vi "Line Configuration Dialog.vi"(8 "error in":errorcluster, 9 "engine configuration in":refnum<class "engine configuration.lvclass">, 10 "tag bus configurable plugin module configuration":refnum<class "Daqmx Module configuration.lvclass">, 11 "Line":T5={"Channel Array"=[], "Physical Channel"="", "Measurement Type"=enum."Digital Input", "Parameters"={"Digital Config"={"Invert Lines?"=FALSE}, "Voltage Config"={"Maximum Value (V)"=5.0, "Minimum Value (V)"=-5.0, "in terminal configuration (V)"=-1, "out terminal configuration (V)"=-1}, "Current Config"={"Maximum Value (A)"=0.02, "Minimum Value (A)"=0.0, "shunt resistor location"=-1, "input terminal configuration (C)"=-1, "external shunt resistor value"=249.0}, "RTD Config"={"Maximum Value (°C)"=100.0, "Minimum Value (°C)"=0.0, "resistance configuration"=2, "r0"=100.0, "current excitation value"=0.0025, "rtd type"=10137, "current excitation source"=10167}, "Thermocouple Config"={"Minimum Value (C)"=0.0, "Maximum Value (C)"=100.0, "thermocouple type"=10072, "cjc source"=10116, "cjc value"=25.0}, "Strain Config"={"Maximum Value"=0.001, "Minimum Value"=-0.001, "bridge information"={"strain configuration"=10183, "lead wire resistance"=0.0, "initial bridge voltage"=0.0, "voltage excitation source"=10200, "voltage excitation value"=2.5}, "strain gage information"={"gage factor"=2.0, "nominal gage resistance"=350.0, "poisson ratio"=0.3}}, "PWM Config"={"Idle State"=FALSE}}} {"Parameters"."Voltage Config"."out terminal configuration (V)" items=["Default"=-1, "RSE"=10083, "Differential"=10106, "Pseudodifferential"=12529]; "Parameters"."Voltage Config"."in terminal configuration (V)" items=["Default"=-1, "RSE"=10083, "NRSE"=10078, "Differential"=10106, "Pseudodifferential"=12529]; "Parameters"."Current Config"."shunt resistor location" items=["default"=-1, "Internal"=10200, "External"=10167]; "Parameters"."Current Config"."input terminal configuration (C)" items=["default"=-1, "RSE"=10083, "NRSE"=10078, "Differential"=10106, "Pseudodifferential"=12529]; "Parameters"."RTD Config"."resistance configuration" items=["2-Wire"=2, "3-Wire"=3, "4-Wire"=4]; "Parameters"."RTD Config"."rtd type" items=["Pt3750"=12481, "Pt3851"=10071, "Pt3911"=12482, "Pt3916"=10069, "Pt3920"=10053, "Pt3928"=12483, "Custom"=10137]; "Parameters"."RTD Config"."current excitation source" items=["Internal"=10200, "External"=10167, "None"=10230]; "Parameters"."Thermocouple Config"."thermocouple type" items=["J"=10072, "K"=10073, "N"=10077, "R"=10082, "S"=10085, "T"=10086, "B"=10047, "E"=10055]; "Parameters"."Thermocouple Config"."cjc source" items=["Built-In"=10200, "Constant Value"=10116, "Channel"=10113]; "Parameters"."Strain Config"."bridge information"."strain configuration" items=["Full Bridge I"=10183, "Full Bridge II"=10184, "Full Bridge III"=10185, "Half Bridge I"=10188, "Half Bridge II"=10189, "Quarter Bridge I"=10271, "Quarter Bridge II"=10272]; "Parameters"."Strain Config"."bridge information"."voltage excitation source" items=["Internal"=10200, "External"=10167, "None"=10230]}) -> (0 "error out":errorcluster, 1 "success":bool, 2 "changed":bool, 3 "Mappings out":T4={"Line"={"Channel Array"=[], "Physical Channel"="", "Measurement Type"=enum."Digital Input", "Parameters"={"Digital Config"={"Invert Lines?"=FALSE}, "Voltage Config"={"Maximum Value (V)"=5.0, "Minimum Value (V)"=-5.0, "in terminal configuration (V)"=-1, "out terminal configuration (V)"=-1}, "Current Config"={"Maximum Value (A)"=0.02, "Minimum Value (A)"=0.0, "shunt resistor location"=-1, "input terminal configuration (C)"=-1, "external shunt resistor value"=249.0}, "RTD Config"={"Maximum Value (°C)"=100.0, "Minimum Value (°C)"=0.0, "resistance configuration"=2, "r0"=100.0, "current excitation value"=0.0025, "rtd type"=10137, "current excitation source"=10167}, "Thermocouple Config"={"Minimum Value (C)"=0.0, "Maximum Value (C)"=100.0, "thermocouple type"=10072, "cjc source"=10116, "cjc value"=25.0}, "Strain Config"={"Maximum Value"=0.001, "Minimum Value"=-0.001, "bridge information"={"strain configuration"=10183, "lead wire resistance"=0.0, "initial bridge voltage"=0.0, "voltage excitation source"=10200, "voltage excitation value"=2.5}, "strain gage information"={"gage factor"=2.0, "nominal gage resistance"=350.0, "poisson ratio"=0.3}}, "PWM Config"={"Idle State"=FALSE}}}, "Maps"=[]} {"Line"."Parameters"."Voltage Config"."out terminal configuration (V)" items=["Default"=-1, "RSE"=10083, "Differential"=10106, "Pseudodifferential"=12529]; "Line"."Parameters"."Voltage Config"."in terminal configuration (V)" items=["Default"=-1, "RSE"=10083, "NRSE"=10078, "Differential"=10106, "Pseudodifferential"=12529]; "Line"."Parameters"."Current Config"."shunt resistor location" items=["default"=-1, "Internal"=10200, "External"=10167]; "Line"."Parameters"."Current Config"."input terminal configuration (C)" items=["default"=-1, "RSE"=10083, "NRSE"=10078, "Differential"=10106, "Pseudodifferential"=12529]; "Line"."Parameters"."RTD Config"."resistance configuration" items=["2-Wire"=2, "3-Wire"=3, "4-Wire"=4]; "Line"."Parameters"."RTD Config"."rtd type" items=["Pt3750"=12481, "Pt3851"=10071, "Pt3911"=12482, "Pt3916"=10069, "Pt3920"=10053, "Pt3928"=12483, "Custom"=10137]; "Line"."Parameters"."RTD Config"."current excitation source" items=["Internal"=10200, "External"=10167, "None"=10230]; "Line"."Parameters"."Thermocouple Config"."thermocouple type" items=["J"=10072, "K"=10073, "N"=10077, "R"=10082, "S"=10085, "T"=10086, "B"=10047, "E"=10055]; "Line"."Parameters"."Thermocouple Config"."cjc source" items=["Built-In"=10200, "Constant Value"=10116, "Channel"=10113]; "Line"."Parameters"."Strain Config"."bridge information"."strain configuration" items=["Full Bridge I"=10183, "Full Bridge II"=10184, "Full Bridge III"=10185, "Half Bridge I"=10188, "Half Bridge II"=10189, "Quarter Bridge I"=10271, "Quarter Bridge II"=10272]; "Line"."Parameters"."Strain Config"."bridge information"."voltage excitation source" items=["Internal"=10200, "External"=10167, "None"=10230]})   [LabVIEW 2015, in "DAQmx Module editor node.lvclass"]
doc: "A dialog for allowing a user to specify the values of a new line."
uses:
  DAQmx Module editor node.lvclass
  module/configuration/Line.ctl
  <vilib>/NI/Tag Bus Module Framework/channel/TBM channel.lvclass
  module/configuration/Measurement Type.ctl
  module/configuration/Parameters.ctl
  Mappings.ctl
  Map.ctl
  <vilib>/NI/Module Execution Interface/Engine Configuration/engine configuration.lvclass
  module/configuration/Daqmx Module configuration.lvclass
  <vilib>/NI/Tag Bus/tag/tag descriptor.lvclass/tag descriptor.ctl
  <vilib>/NI/Configuration Framework/serializable configuration/NISE_CEF_serializable configuration.lvclass/NISE_CEF_serializable configuration.ctl
  <vilib>/NI/Tag Bus Module Framework/channel/TBM channel.lvclass/TBM channel.ctl
  <vilib>/NI/Tag Bus/tag/write metadata.vi
  <vilib>/NI/Tag Bus/tag/write tag name.vi
  <vilib>/NI/Tag Bus/tag/write data type.vi
  <vilib>/NI/Tag Bus Module Framework/channel/Write channel classification.vi
  <vilib>/NI/Configuration Framework/serializable configuration/Read UID.vi
  <vilib>/Utility/LVClass/Get LV Class Name.vi
  <vilib>/NI/Configuration Framework/error generator/NISE_error generator.vi
  <vilib>/NI/Tag Bus/tag/tag descriptor.lvclass
  <vilib>/NI/DCAF UI Toolkit/Controls/DCAF UI Elements.lvlib
panel:
  in  "DAQmx Physical Channel":tag
  out "Tab Control":T1(tab)
  in  "Invert Lines?":bool
  in  "out terminal configuration (V)":i32(ring)=-1 items=["Default"=-1, "RSE"=10083, "Differential"=10106, "Pseudodifferential"=12529]
  in  "in terminal configuration (V)":i32(ring)=-1 items=["Default"=-1, "RSE"=10083, "NRSE"=10078, "Differential"=10106, "Pseudodifferential"=12529]
  in  "Maximum Value (V)":dbl=5.0 format="%0.2f"
  in  "Minimum Value (V)":dbl=-5.0 format="%0.2f"
  in  "input terminal configuration (C)":i32(ring)=-1 items=["default"=-1, "RSE"=10083, "NRSE"=10078, "Differential"=10106, "Pseudodifferential"=12529]
  in  "shunt resistor location":i32(ring)=-1 items=["default"=-1, "Internal"=10200, "External"=10167]
  in  "external shunt resistor value":dbl=249.0 format="%0.2f"
  in  "Maximum Value (A)":dbl=0.02 format="%0.5f"
  in  "Minimum Value (A)":dbl format="%0.5f"
  in  "r0":dbl=100.0 format="%0.2f"
  in  "resistance configuration":i32(ring)=2 items=["2-Wire"=2, "3-Wire"=3, "4-Wire"=4]
  in  "Maximum Value (°C)":dbl=100.0 format="%0.2f"
  in  "Minimum Value (°C)":dbl format="%0.2f"
  in  "rtd type":i32(ring)=12481 items=["Pt3750"=12481, "Pt3851"=10071, "Pt3911"=12482, "Pt3916"=10069, "Pt3920"=10053, "Pt3928"=12483, "Custom"=10137]
  in  "current excitation value":dbl=0.0025 format="%0.5f"
  in  "current excitation source":i32(ring)=10167 items=["Internal"=10200, "External"=10167, "None"=10230]
  in  "strain gage information":T2={"gage factor"=2.0, "nominal gage resistance"=350.0, "poisson ratio"=0.3} {"poisson ratio" format="%0.2f"; "nominal gage resistance" format="%0.2f"; "gage factor" format="%0.2f"}
  in  "bridge information":T3={"strain configuration"=10183, "lead wire resistance"=0.0, "initial bridge voltage"=0.0, "voltage excitation source"=10200, "voltage excitation value"=2.5} {"initial bridge voltage" format="%0.2f"; "voltage excitation source" items=["Internal"=10200, "External"=10167, "None"=10230]; "voltage excitation value" format="%0.2f"; "lead wire resistance" format="%0.2f"; "strain configuration" items=["Full Bridge I"=10183, "Full Bridge II"=10184, "Full Bridge III"=10185, "Half Bridge I"=10188, "Half Bridge II"=10189, "Quarter Bridge I"=10271, "Quarter Bridge II"=10272]}
  in  "Minimum Value":dbl=-0.001 format="%0.7f"
  in  "Maximum Value":dbl=0.001 format="%0.7f"
  in  "cjc value":dbl=25.0 format="%0.2f"
  in  "thermocouple type":i32(ring)=10072 items=["J"=10072, "K"=10073, "N"=10077, "R"=10082, "S"=10085, "T"=10086, "B"=10047, "E"=10055]
  in  "Maximum Value (C)":dbl=100.0 format="%0.2f"
  in  "Minimum Value (C)":dbl format="%0.2f"
  in  "cjc source":i32(ring)=10116 items=["Built-In"=10200, "Constant Value"=10116, "Channel"=10113]
  in  "Duty Cycle":i32(listbox)
  in  "Frequency":i32(listbox)
  in  "Idle State":bool
  in  "Measurement Type":i32(listbox)
  out "errors":string
  in  "Tag":i32(listbox)
  in  "Description":string
  in  "cancel":bool
  in  "ok":bool
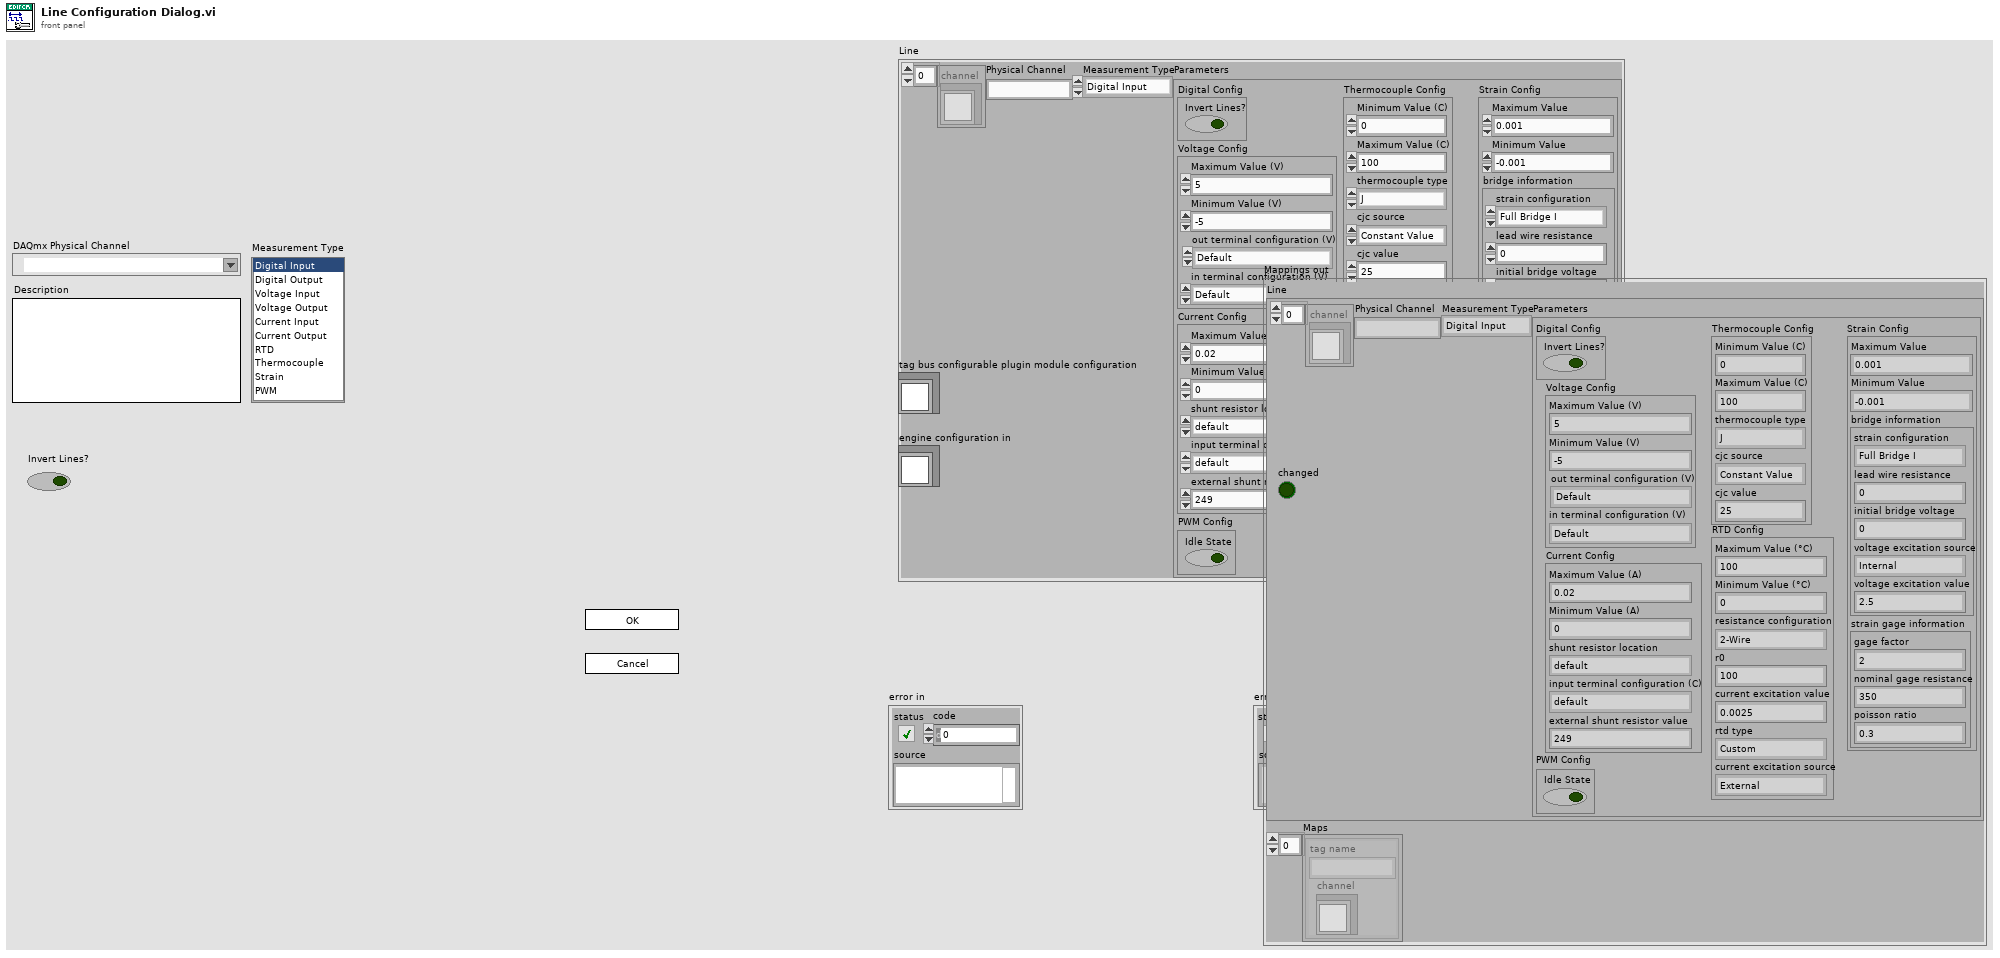
[diagram p1: front panel]
types:
  T1 = enum32{"Digital", "Voltage", "Current", "RTD", "Strain", "Thermocouple", "PWM"}
  T2 = cluster{"gage factor":dbl, "nominal gage resistance":dbl, "poisson ratio":dbl}
  T3 = cluster{"strain configuration":i32, "lead wire resistance":dbl, "initial bridge voltage":dbl, "voltage excitation source":i32, "voltage excitation value":dbl}
  T4 = typedef "DAQmx Module editor node.lvclass/Mappings.ctl" = cluster{"Line":T5, "Maps":T8[]}
  T5 = typedef "DAQmx Module Configuration.lvclass/Line.ctl" = cluster{"Channel Array":refnum<class "TBM channel.lvclass">[], "Physical Channel":string, "Measurement Type":T6, "Parameters":T7}
  T6 = typedef "DAQmx Module Configuration.lvclass/Measurement Type.ctl" = enum16{"Digital Input", "Digital Output", "Voltage Input", "Voltage Output", "Current Input", "Current Output", "RTD", "Thermocouple", "Strain", "PWM"}
  T7 = typedef "DAQmx Module Configuration.lvclass/Parameters.ctl" = cluster{"Digital Config":cluster{"Invert Lines?":bool}, "Voltage Config":cluster{"Maximum Value (V)":dbl, "Minimum Value (V)":dbl, "in terminal configuration (V)":i32, "out terminal configuration (V)":i32}, "Current Config":cluster{"Maximum Value (A)":dbl, "Minimum Value (A)":dbl, "shunt resistor location":i32, "input terminal configuration (C)":i32, "external shunt resistor value":dbl}, "RTD Config":cluster{"Maximum Value (°C)":dbl, "Minimum Value (°C)":dbl, "resistance configuration":i32, "r0":dbl, "current excitation value":dbl, "rtd type":i32, "current excitation source":i32}, "Thermocouple Config":cluster{"Minimum Value (C)":dbl, "Maximum Value (C)":dbl, "thermocouple type":i32, "cjc source":i32, "cjc value":dbl}, "Strain Config":cluster{"Maximum Value":dbl, "Minimum Value":dbl, "bridge information":cluster{"strain configuration":i32, "lead wire resistance":dbl, "initial bridge voltage":dbl, "voltage excitation source":i32, "voltage excitation value":dbl}, "strain gage information":cluster{"gage factor":dbl, "nominal gage resistance":dbl, "poisson ratio":dbl}}, "PWM Config":cluster{"Idle State":bool}}
  T8 = typedef "DAQmx Module editor node.lvclass/Map.ctl" = cluster{"channel":refnum<class "TBM channel.lvclass">, "tag name":string}
  T9 = enum8{"Enabled", "Disabled", "Disabled and Grayed Out"}
  T10 = enum32{"Digital", "Voltage", "Current", "RTD", "Strain", "Thermocouple"}
  T11 = typedef "TBM channel.lvclass/channel classification.ctl" = enum16{"input data", "output data", "processing parameter", "processing result"}
  T12 = typedef "tag bus.lvlib/tag descriptor.lvclass/Data Type.ctl" = enum16{"Double", "Single", "I64", "I32", "I16", "I8", "U64", "U32", "U16", "U8", "Boolean", "String", "Array of Double", "Array of Single", "Array of I64", "Array of I32", "Array of I16", "Array of I8", "Array of U64", "Array of U32", "Array of U16", "Array of U8", "Array of Boolean", "Array of String"}
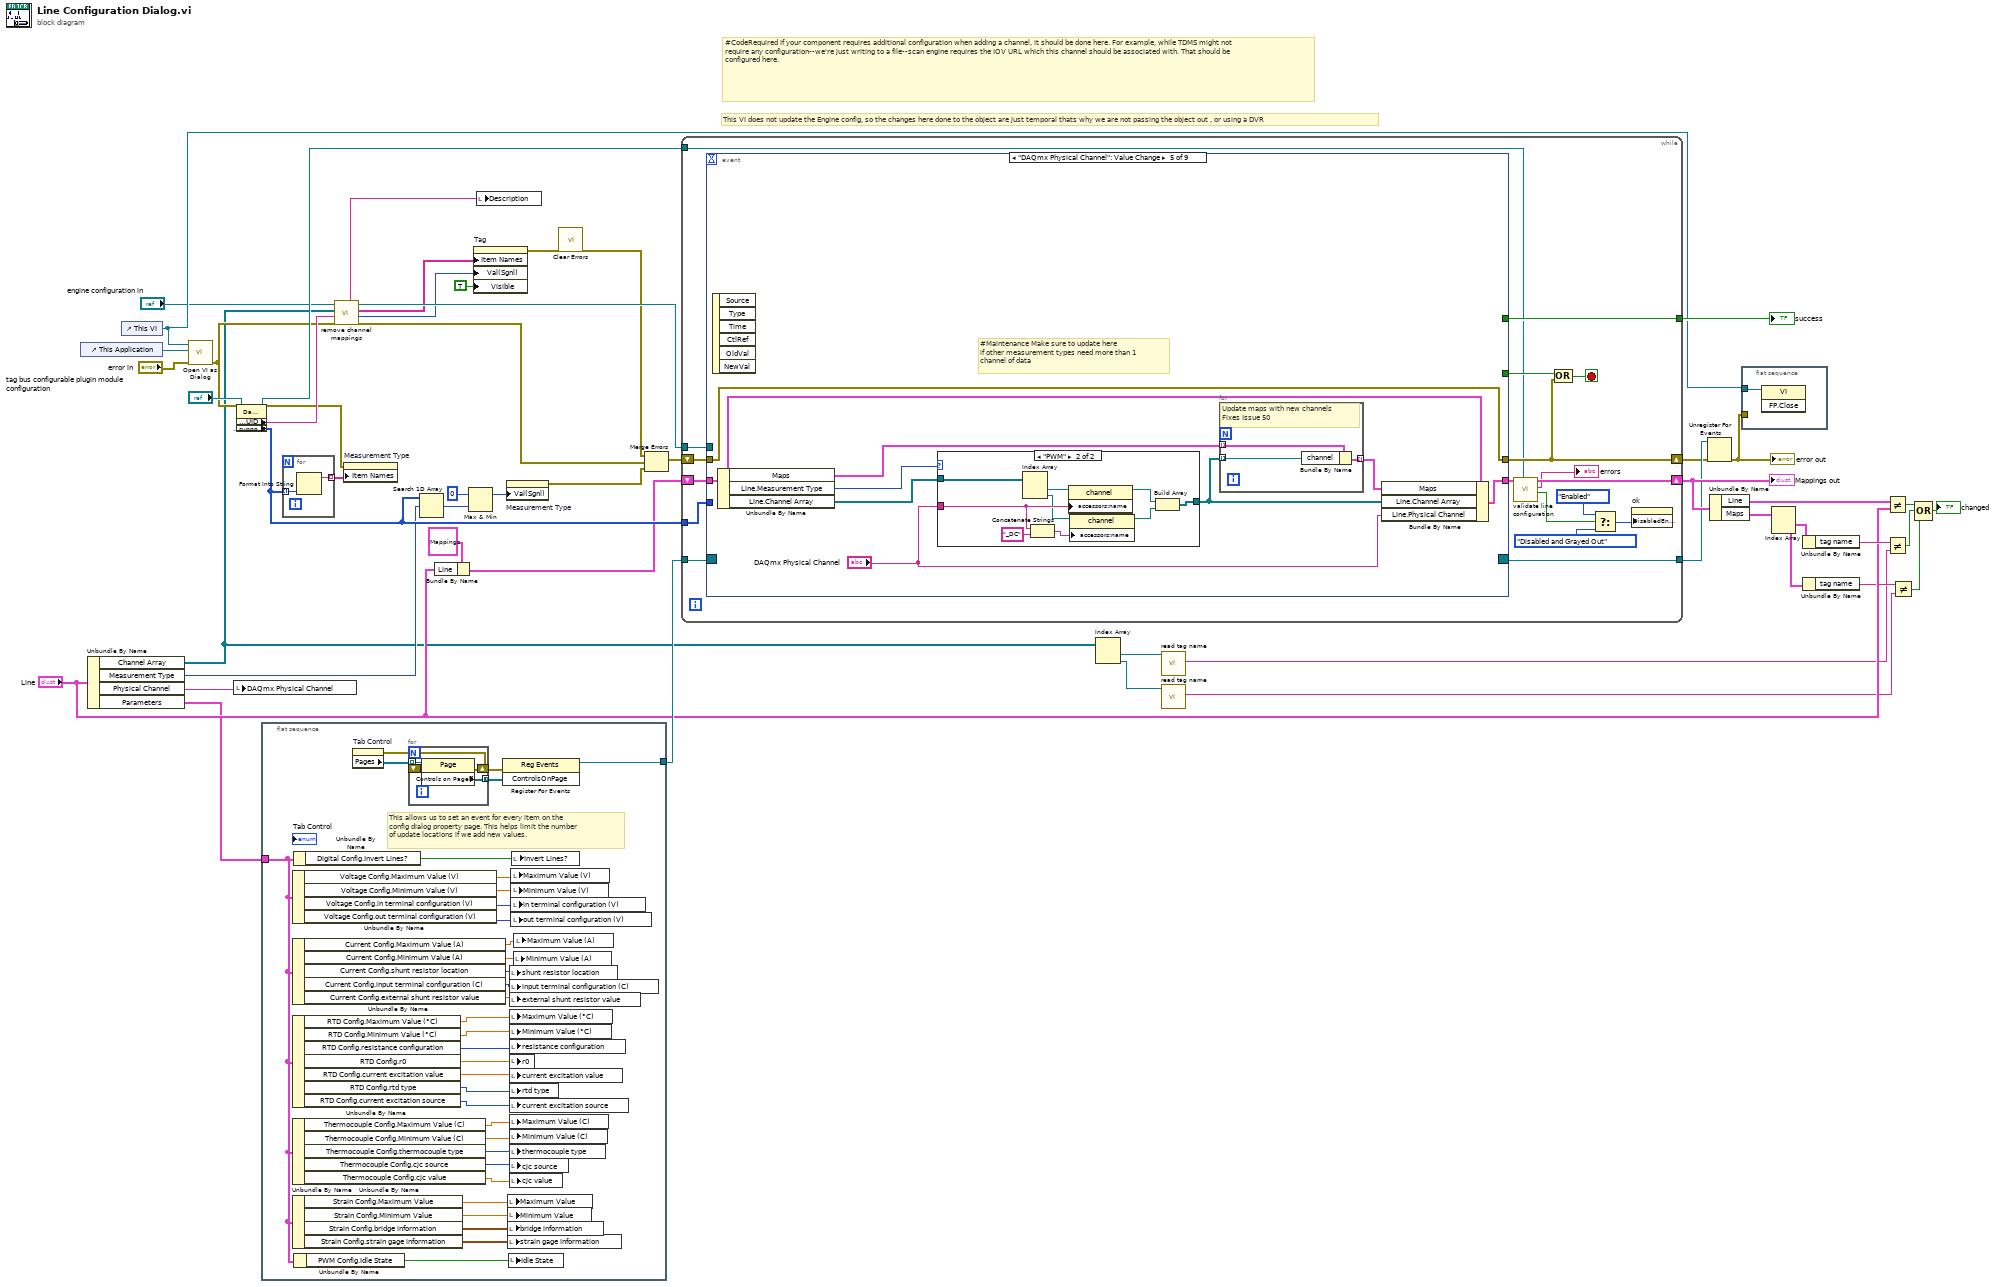
[diagram p0: block diagram]
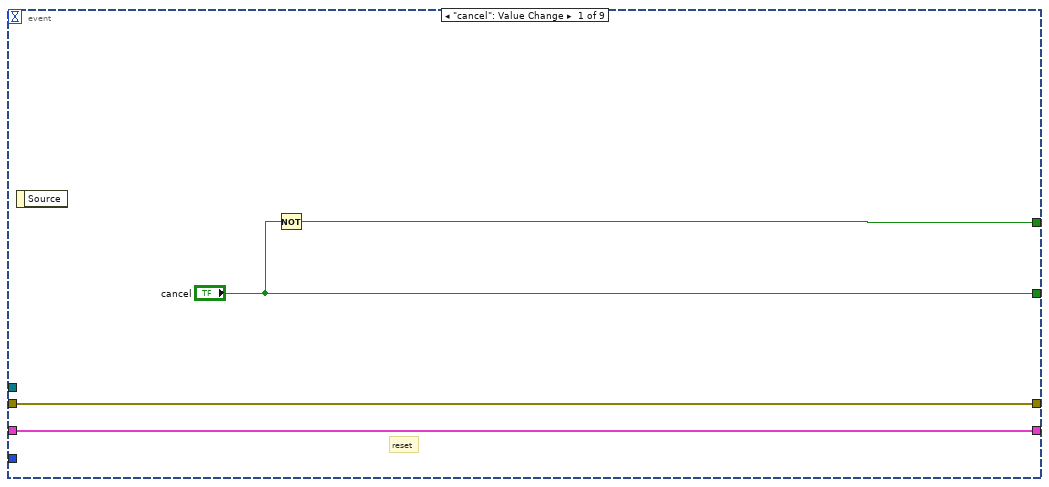
[diagram p2: hidden frame]
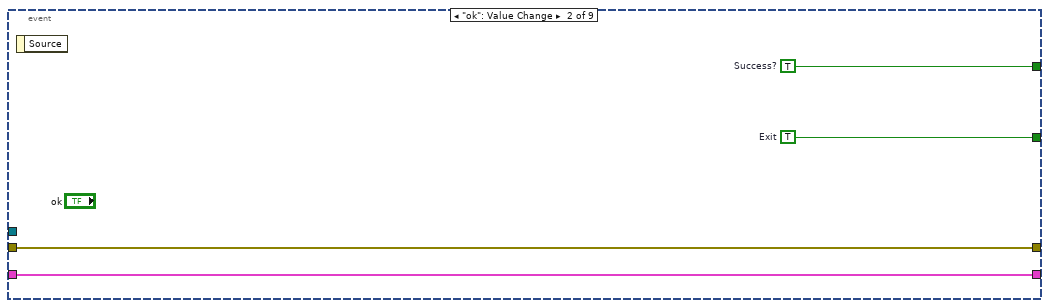
[diagram p3: hidden frame]
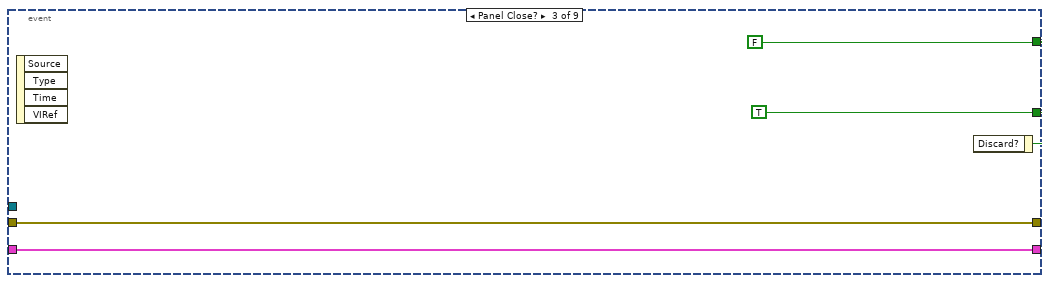
[diagram p4: hidden frame]
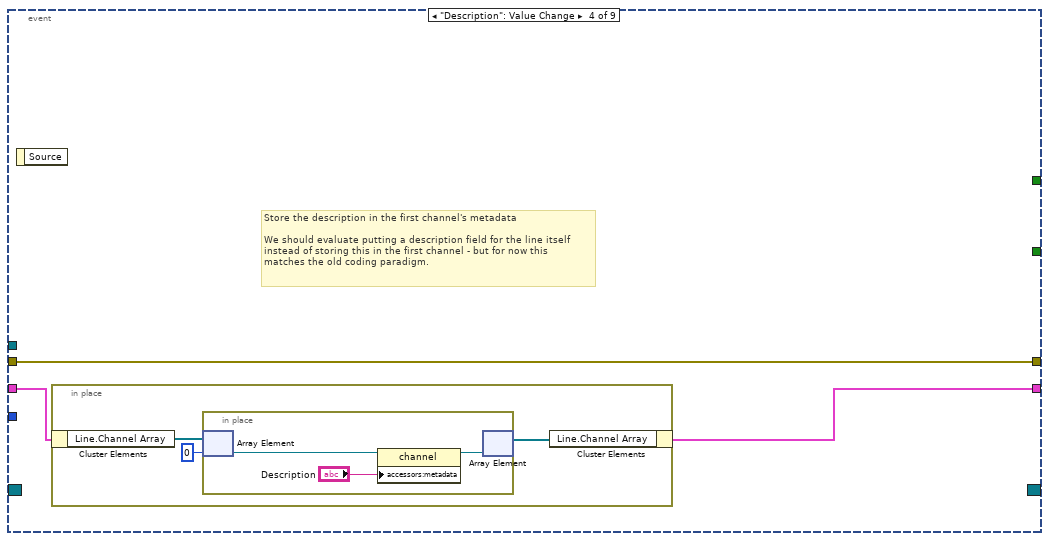
[diagram p5: hidden frame]
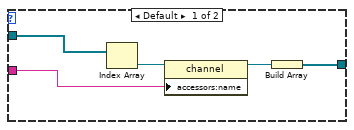
[diagram p6: hidden frame]
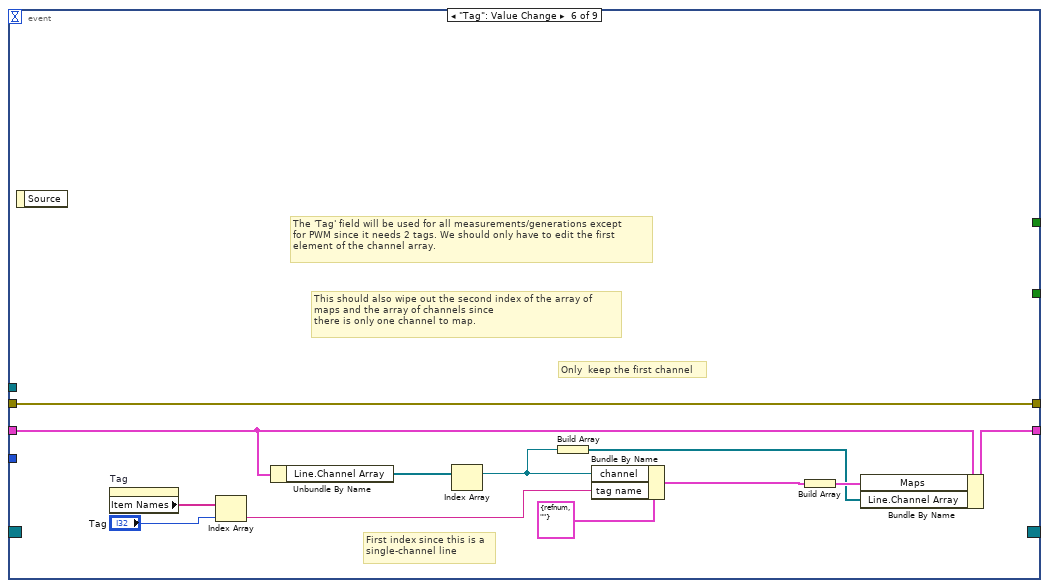
[diagram p7: hidden frame]
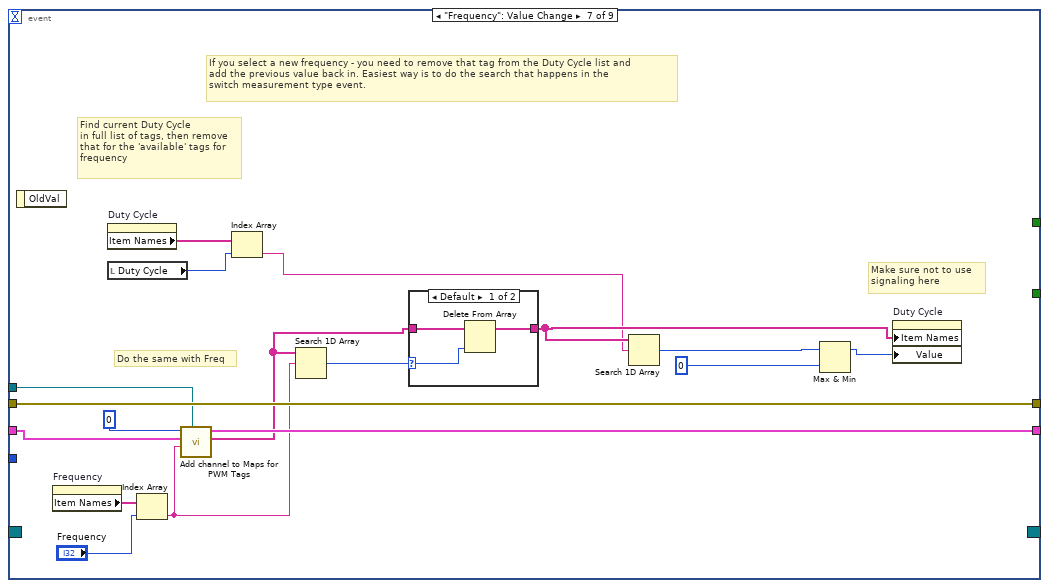
[diagram p8: hidden frame]
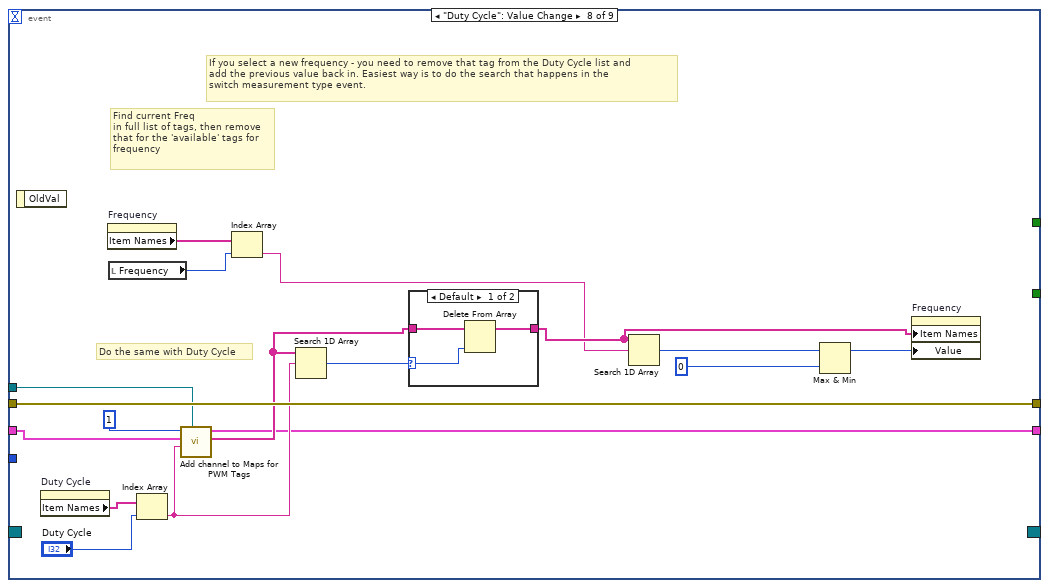
[diagram p10: hidden frame]
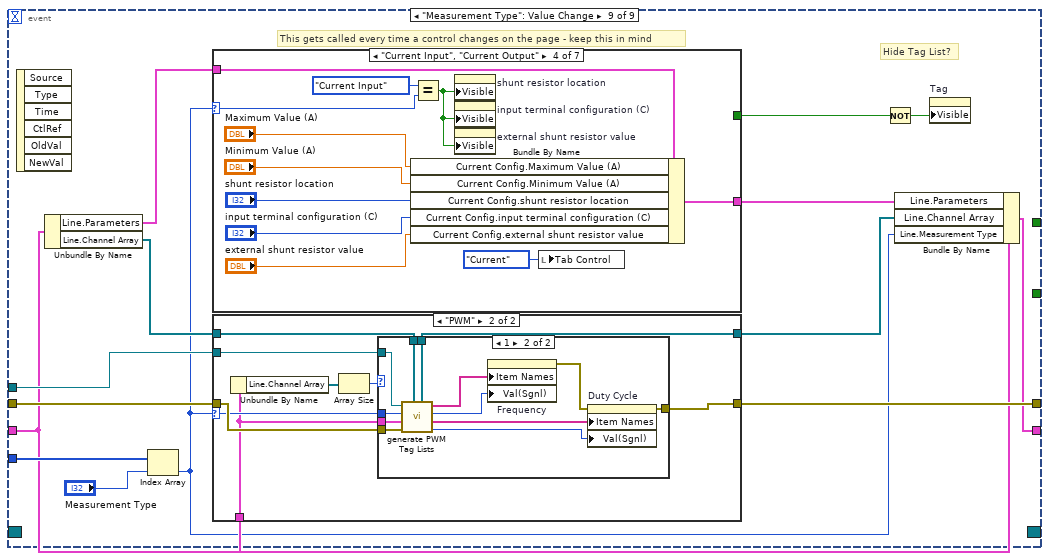
[diagram p12: hidden frame]
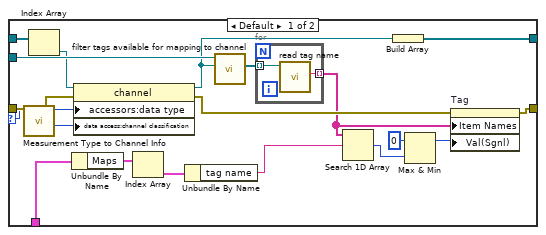
[diagram p13: hidden frame]
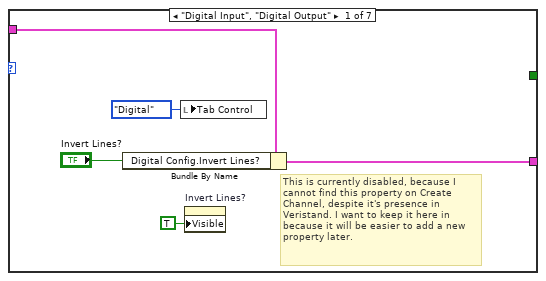
[diagram p15: hidden frame]
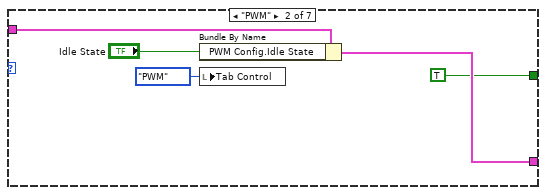
[diagram p16: hidden frame]
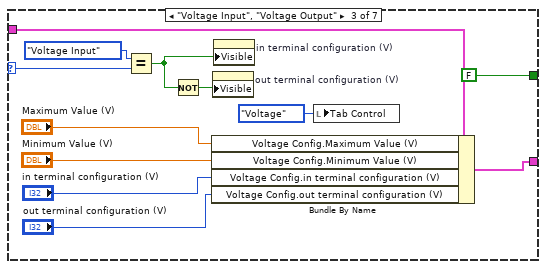
[diagram p17: hidden frame]
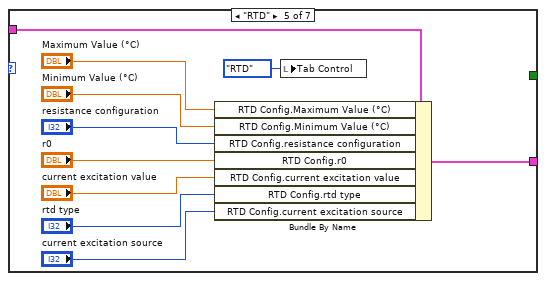
[diagram p18: hidden frame]
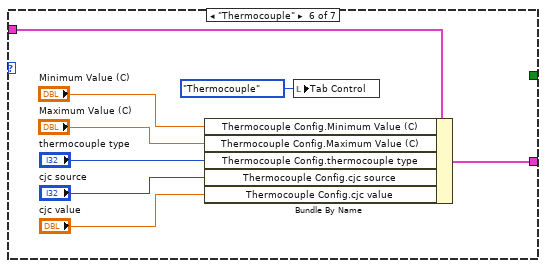
[diagram p19: hidden frame]
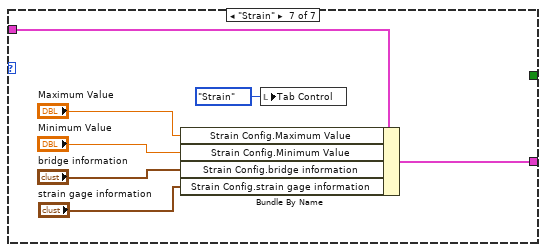
[diagram p20: hidden frame]
diagram:
  # "This VI does not update the Engine config, so the changes here done to the object are just temporal thats why we are not passing the object out , or using a DVR"
  # "#CodeRequired If your component requires additional configuration when adding a channel, it should be done here. For example, while TDMS might not require any configuration--we're just writing to a file--scan engine requires the IOV URL which this channel should be associated with. That should be configured here."
  n1 = control-ref of="This Application"() -> (w44:refnum<vi>)
  n2 = Unbundle By Name("Line") -> ("Channel Array"=w8:refnum<class "TBM channel.lvclass">[], "Measurement Type"=w27:T6, "Physical Channel"=w26:string, "Parameters"=w20:T7)
  n3 = control-ref of="This VI"() -> (w34:refnum<vi>)
  n4 = call <vilib>:"Open VI as Dialog.vi"("error in (no error)"="error in", "This Application"=w44, "VI in"=w34) -> ("error out"=w16:errorcluster)  [unwired: 8 in]
  n5 = local write "DAQmx Physical Channel"(w26) -> ()
  n6 = property class="Daqmx Module configuration"(reference="tag bus configurable plugin module configuration", error in=w16) -> (reference out=w41:refnum<class "Daqmx Module configuration.lvclass">, error out=w32:errorcluster, "Properties:UID"=w42:string, "Customize:Properties:supported measurement types"=w28:T6[])
  n7 = flat-sequence {
    tunnel: [w84] -> w22
    tunnel: w20 -> [w53]
    frame #0 {
      # "This allows us to set an event for every item on the \nconfig dialog property page. This helps limit the number \nof update locations if we add new values."
      n8 = Unbundle By Name(w53) -> ("Voltage Config.Maximum Value (V)"=w82:dbl, "Voltage Config.Minimum Value (V)"=w81:dbl, "Voltage Config.in terminal configuration (V)"=w80:i32, "Voltage Config.out terminal configuration (V)"=w58:i32)
      n9 = Unbundle By Name(w53) -> ("Current Config.Maximum Value (A)"=w71:dbl, "Current Config.Minimum Value (A)"=w72:dbl, "Current Config.shunt resistor location"=w74:i32, "Current Config.input terminal configuration (C)"=w83:i32, "Current Config.external shunt resistor value"=w73:dbl)
      n10 = Unbundle By Name(w53) -> ("RTD Config.Maximum Value (°C)"=w70:dbl, "RTD Config.Minimum Value (°C)"=w69:dbl, "RTD Config.resistance configuration"=w68:i32, "RTD Config.r0"=w67:dbl, "RTD Config.current excitation value"=w66:dbl, "RTD Config.rtd type"=w65:i32, "RTD Config.current excitation source"=w64:i32)
      n11 = Unbundle By Name(w53) -> ("Thermocouple Config.Maximum Value (C)"=w61:dbl, "Thermocouple Config.Minimum Value (C)"=w62:dbl, "Thermocouple Config.thermocouple type"=w63:i32, "Thermocouple Config.cjc source"=w60:i32, "Thermocouple Config.cjc value"=w59:dbl)
      n12 = Unbundle By Name(w53) -> ("Strain Config.Maximum Value"=w75:dbl, "Strain Config.Minimum Value"=w76:dbl, "Strain Config.bridge information"=w77:T3, "Strain Config.strain gage information"=w78:T2)
      n13 = Unbundle By Name(w53) -> ("Digital Config.Invert Lines?"=w79:bool)
      n14 = Unbundle By Name(w53) -> ("PWM Config.Idle State"=w52:bool)
      n15 = property on="Tab Control" class="TabCtl (strict)"() -> (error out=w56:errorcluster, "Pages"=w57:refnum<vi>[])  [unwired: 2 in, 1 out]
      n16 = for {
        tunnel: w57 -> [w88] mode=indexing
        tunnel: [w85] -> w54 mode=concatenating
        shift-right: [w86] -> w55
        shift-left: w56 -> [w87]
        n17 = property class="Page"(reference=w88, error in=w87) -> (error out=w86:errorcluster, "Controls on Page[]"=w85:refnum<vi>[])  [unwired: 1 out]
      }
      n18 = register-events(error in=w55, w54) -> (reference out=w84:refnum<event-registration>)  [unwired: 1 in, 1 out]
      n19 = local write "Maximum Value"(w75) -> ()
      n20 = local write "Minimum Value"(w76) -> ()
      n21 = local write "bridge information"(w77) -> ()
      n22 = local write "strain gage information"(w78) -> ()
      n23 = local write "Idle State"(w52) -> ()
      n24 = local write "shunt resistor location"(w74) -> ()
      n25 = local write "input terminal configuration (C)"(w83) -> ()
      n26 = local write "external shunt resistor value"(w73) -> ()
      n27 = local write "Maximum Value (°C)"(w70) -> ()
      n28 = local write "Minimum Value (°C)"(w69) -> ()
      n29 = local write "resistance configuration"(w68) -> ()
      n30 = local write "r0"(w67) -> ()
      n31 = local write "current excitation value"(w66) -> ()
      n32 = local write "rtd type"(w65) -> ()
      n33 = local write "current excitation source"(w64) -> ()
      n34 = local write "Maximum Value (C)"(w61) -> ()
      n35 = local write "Minimum Value (C)"(w62) -> ()
      n36 = local write "thermocouple type"(w63) -> ()
      n37 = local write "cjc source"(w60) -> ()
      n38 = local write "cjc value"(w59) -> ()
      n39 = local write "Maximum Value (V)"(w82) -> ()
      n40 = local write "Minimum Value (V)"(w81) -> ()
      n41 = local write "in terminal configuration (V)"(w80) -> ()
      n42 = local write "out terminal configuration (V)"(w58) -> ()
      n43 = local write "Invert Lines?"(w79) -> ()
      n44 = local write "Minimum Value (A)"(w72) -> ()
      n45 = local write "Maximum Value (A)"(w71) -> ()
    }
  }
  n46 = for {
    tunnel: w28 -> [w90] mode=indexing
    tunnel: [w89] -> w33 mode=indexing
    n47 = Format Into String(w90) -> (resulting string=w89:string)  [unwired: 3 in, 1 out]
  }
  n48 = call "remove channel mappings.vi"("error in (no error)"=w16, "Properties:UID"=w42, "Channel Array"=w8, "engine configuration in"="engine configuration in") -> ("error out"=w10:errorcluster, "Numeric"=w23:i32, "Array"=w24:string[], "engine configuration out"=w50:refnum<class "engine configuration.lvclass">, "accessors:metadata"=w49:string)  [unwired: 2 in, 1 out]
  n49 = property on="Measurement Type" class="LstBox (strict)"(error in=w32, "Item Names"=w33) -> ()  [unwired: 1 in, 2 out]
  n50 = Search 1D Array(1D array=w28, element=w27) -> (index of element=w29:i32)  [unwired: 1 in]
  n51 = Bundle By Name(cluster=T4 {"Line"={"Channel Array"=[], "Physical Channel"="", "Measurement Type"=enum."Digital Input", "Parameters"={"Digital Config"={"Invert Lines?"=FALSE}, "Voltage Config"={"Maximum Value (V)"=5.0, "Minimum Value (V)"=-5.0, "in terminal configuration (V)"=-1, "out terminal configuration (V)"=-1}, "Current Config"={"Maximum Value (A)"=0.02, "Minimum Value (A)"=0.0, "shunt resistor location"=-1, "input terminal configuration (C)"=-1, "external shunt resistor value"=249.0}, "RTD Config"={"Maximum Value (°C)"=100.0, "Minimum Value (°C)"=0.0, "resistance configuration"=2, "r0"=100.0, "current excitation value"=0.0025, "rtd type"=10137, "current excitation source"=10167}, "Thermocouple Config"={"Minimum Value (C)"=0.0, "Maximum Value (C)"=100.0, "thermocouple type"=10072, "cjc source"=10116, "cjc value"=25.0}, "Strain Config"={"Maximum Value"=0.001, "Minimum Value"=-0.001, "bridge information"={"strain configuration"=10183, "lead wire resistance"=0.0, "initial bridge voltage"=0.0, "voltage excitation source"=10200, "voltage excitation value"=2.5}, "strain gage information"={"gage factor"=2.0, "nominal gage resistance"=350.0, "poisson ratio"=0.3}}, "PWM Config"={"Idle State"=FALSE}}}, "Maps"=[]} ("Mappings out"), "Line"="Line") -> (w25:T4)
  n52 = Max & Min(x=0 ("f"), y=w29) -> (max(x,y)=w31:i32)  [unwired: 1 out]
  n53 = property on="Tag" class="LstBox (strict)"("Item Names"=w24, "Val(Sgnl)"=w23, "Visible"=TRUE) -> (error out=w14:errorcluster)  [unwired: 2 in, 1 out]
  n54 = local write "Description"(w49) -> ()
  n55 = property on="Measurement Type" class="LstBox (strict)"("Val(Sgnl)"=w31) -> (error out=w11:errorcluster)  [unwired: 2 in, 1 out]
  n56 = call <vilib>:"Clear Errors.vi"("error in (no error)"=w14) -> ("error out"=w12:errorcluster)  [unwired: 5 in, 1 out]
  n57 = Merge Errors(w12, w10, w11) -> (w13:errorcluster)
  n58 = while {
    shift-right: [w100] -> w18
    shift-left: w13 -> [w107]
    tunnel: [w106] -> w51
    shift-right: [w101] -> w45
    shift-left: w25 -> [w103]
    tunnel: w50 -> [w108]
    tunnel: w41 -> [w93]
    tunnel: w28 -> [w95]
    tunnel: w22 -> [w94]
    tunnel: [w92] -> w19
    stop <- w104 stop-if-true
    n59 = event shown="[4] \"DAQmx Physical Channel\": Value Change" {
      selector: w94 -> [_ _ _ _ _ _ _ _ _]
      dyn-events: [_ _ _ _ _ _ _ _ _] -> w92
      timeout: _ -> [_ _ _ _ _ _ _ _ _]
      tunnel: w108 -> [_ _ _ _ _ _ w178 w202 w222]
      tunnel: w107 -> [w112 w116 w120 w123 w135 w167 w184 w205 w214]
      tunnel: [w112 w116 w120 w123 w135 w167 w184 w205 w223] -> w100
      tunnel: [w111 w113 FALSE _ _ _ _ _ _] -> w106
      tunnel: ["cancel" w114 w118 _ _ _ _ _ _] -> w105
      tunnel: w103 -> [w109 w115 w117 w122 w137 w162 w180 w203 w211]
      tunnel: [w109 w115 w117 w121 w138 w159 w179 w189 w219] -> w102
      tunnel: w95 -> [_ _ _ _ _ _ _ _ w220]
      event "cancel": Value Change {
        # "reset"
        n60 = event-data() -> ()  [unwired: 1 in, 1 out]
        n61 = Not(x="cancel") -> (.not. x?=w111:bool)
      }
      event "ok": Value Change {
        w113 = TRUE  # Success?
        w114 = TRUE  # Exit
        n62 = event-data() -> ()  [unwired: 1 in, 1 out]
      }
      event Panel Close? {
        w118 = TRUE ("cancel")
        n63 = event-data() -> ()  [unwired: 1 in, 4 out]
        n64 = event-data("Discard?"=w118) -> ()  [unwired: 1 in, 1 out]
      }
      event "Description": Value Change {
        # "Store the description in the first channel's metadata\n\nWe should evaluate putting a description field for the line itself\ninstead of storing this in the first channel - but for now this\nmatches the old coding paradigm."
        n65 = event-data() -> ()  [unwired: 1 in, 1 out]
        n66 = in-place {
          n67 = in-place-cluster #1(w122) -> ("Line.Channel Array"=w126:refnum<class "TBM channel.lvclass">[])
          n68 = in-place {
            n69 = in-place-array #2(w126, 0) -> (w128:refnum<class "TBM channel.lvclass">)
            n70 = property class="channel"(reference=w128, "accessors:metadata"="Description") -> (reference out=w127:refnum<class "TBM channel.lvclass">)  [unwired: 1 in, 1 out]
            n71 = in-place-array #2(w127) -> (w124:refnum<class "TBM channel.lvclass">[])  [unwired: 1 out]
          }
          n72 = in-place-cluster #1("Line.Channel Array"=w124) -> (w121:T4)
        }
      }
      event "DAQmx Physical Channel": Value Change {
        # "#Maintenance Make sure to update here\nif other measurement types need more than 1\nchannel of data"
        n73 = event-data() -> ()  [unwired: 1 in, 6 out]
        n74 = Unbundle By Name(w137) -> ("Maps"=w132:T8[], "Line.Measurement Type"=w133:T6, "Line.Channel Array"=w134:refnum<class "TBM channel.lvclass">[])
        n75 = case shown="\"PWM\"" w133 {
          tunnel: "DAQmx Physical Channel" -> [w146 w153]
          tunnel: w134 -> [w145 w155]
          tunnel: [w142 w147] -> w130
          frame Default {
            n76 = Index Array(array=w145) -> (element=w144:refnum<class "TBM channel.lvclass">)  [unwired: 1 in]
            n77 = property class="channel"(reference=w144, "accessors:name"=w146) -> (reference out=w143:refnum<class "TBM channel.lvclass">)  [unwired: 1 in, 1 out]
            n78 = Build Array(w143) -> (w142:refnum<class "TBM channel.lvclass">[])
          }
          frame "PWM" {
            n79 = Index Array(array=w155) -> (element #1=w154:refnum<class "TBM channel.lvclass">, element #2=w150:refnum<class "TBM channel.lvclass">)  [unwired: 2 in]
            n80 = Concatenate Strings(w153, "_DC" ("string")) -> (w151:string)
            n81 = property class="channel"(reference=w154, "accessors:name"=w153) -> (reference out=w149:refnum<class "TBM channel.lvclass">)  [unwired: 1 in, 1 out]
            n82 = property class="channel"(reference=w150, "accessors:name"=w151) -> (reference out=w148:refnum<class "TBM channel.lvclass">)  [unwired: 1 in, 1 out]
            n83 = Build Array(w149, w148) -> (w147:refnum<class "TBM channel.lvclass">[])
          }
        }
        n84 = for {
          tunnel: w132 -> [w141] mode=indexing
          tunnel: [w140] -> w131 mode=indexing
          tunnel: w130 -> [w139] mode=indexing
          # "Update maps with new channels\nFixes Issue 50"
          n85 = Bundle By Name(cluster=w141, "channel"=w139) -> (w140:T8)
        }
        n86 = Bundle By Name(cluster=w137, "Maps"=w131, "Line.Channel Array"=w130, "Line.Physical Channel"="DAQmx Physical Channel") -> (w138:T4)
      }
      event "Tag": Value Change {
        # "Only  keep the first channel"
        # "This should also wipe out the second index of the array of \nmaps and the array of channels since\nthere is only one channel to map."
        # "First index since this is a \nsingle-channel line"
        # "The 'Tag' field will be used for all measurements/generations except\nfor PWM since it needs 2 tags. We should only have to edit the first \nelement of the channel array."
        n87 = event-data() -> ()  [unwired: 1 in, 1 out]
        n88 = property on="Tag" class="LstBox (strict)"() -> ("Item Names"=w165:string[])  [unwired: 2 in, 2 out]
        n89 = Index Array(array=w165, index="Tag") -> (element=w158:string)
        n90 = Unbundle By Name(w162) -> ("Line.Channel Array"=w163:refnum<class "TBM channel.lvclass">[])
        n91 = Index Array(array=w163) -> (element=w157:refnum<class "TBM channel.lvclass">)  [unwired: 1 in]
        n92 = Build Array(w157) -> (w156:refnum<class "TBM channel.lvclass">[])
        n93 = Bundle By Name(cluster=T8 {"channel"=refnum, "tag name"=""} ("Map"), "channel"=w157, "tag name"=w158) -> (w161:T8)
        n94 = Build Array(w161) -> (w160:T8[])
        n95 = Bundle By Name(cluster=w162, "Maps"=w160, "Line.Channel Array"=w156) -> (w159:T4)
      }
      event "Frequency": Value Change {
        # "Make sure not to use \nsignaling here"
        # "Do the same with Freq"
        # "Find current Duty Cycle\nin full list of tags, then remove\nthat for the 'available' tags for \nfrequency"
        # "If you select a new frequency - you need to remove that tag from the Duty Cycle list and \nadd the previous value back in. Easiest way is to do the search that happens in the\nswitch measurement type event."
        n96 = event-data() -> ()  [unwired: 1 in, 1 out]
        n97 = property on="Frequency" class="LstBox (strict)"() -> ("Item Names"=w182:string[])  [unwired: 2 in, 2 out]
        n98 = property on="Duty Cycle" class="LstBox (strict)"() -> ("Item Names"=w177:string[])  [unwired: 2 in, 2 out]
        n99 = local read "Duty Cycle"() -> (w176:i32)
        n100 = Index Array(array=w182, index="Frequency") -> (element=w170:string)
        n101 = call "Add channel to Maps for PWM Tags.vi"("engine configuration in"=w178, "Tag Name In"=w170, "Mappings in"=w180, "Index"=0) -> ("Full Tag List"=w169:string[], "Mappings out"=w179:T4)  [unwired: 6 in]
        n102 = Index Array(array=w177, index=w176) -> (element=w168:string)
        n103 = Search 1D Array(1D array=w169, element=w170) -> (index of element=w175:i32)  [unwired: 1 in]
        n104 = case shown="Default" w175 {
          selector: w175 -> [w186 _]
          tunnel: w169 -> [w187 w188]
          tunnel: [w185 w188] -> w174
          frame Default {
            n105 = Delete From Array(array=w187, index=w186) -> (array with subset deleted=w185:string[])  [unwired: 1 in, 1 out]
          }
          frame -1 {
          }
        }
        n106 = Search 1D Array(1D array=w174, element=w168) -> (index of element=w173:i32)  [unwired: 1 in]
        n107 = Max & Min(x=w173, y=0) -> (max(x,y)=w172:i32)  [unwired: 1 out]
        n108 = property on="Duty Cycle" class="LstBox (strict)"("Item Names"=w174, "Value"=w172) -> ()  [unwired: 2 in, 2 out]
      }
      event "Duty Cycle": Value Change {
        # "Do the same with Duty Cycle"
        # "Find current Freq\nin full list of tags, then remove\nthat for the 'available' tags for \nfrequency"
        # "If you select a new frequency - you need to remove that tag from the Duty Cycle list and \nadd the previous value back in. Easiest way is to do the search that happens in the\nswitch measurement type event."
        n109 = event-data() -> ()  [unwired: 1 in, 1 out]
        n110 = property on="Duty Cycle" class="LstBox (strict)"() -> ("Item Names"=w197:string[])  [unwired: 2 in, 2 out]
        n111 = property on="Frequency" class="LstBox (strict)"() -> ("Item Names"=w201:string[])  [unwired: 2 in, 2 out]
        n112 = local read "Frequency"() -> (w200:i32)
        n113 = Index Array(array=w197, index="Duty Cycle") -> (element=w193:string)
        n114 = call "Add channel to Maps for PWM Tags.vi"("engine configuration in"=w202, "Tag Name In"=w193, "Mappings in"=w203, "Index"=1) -> ("Full Tag List"=w191:string[], "Mappings out"=w189:T4)  [unwired: 6 in]
        n115 = Index Array(array=w201, index=w200) -> (element=w190:string)
        n116 = Search 1D Array(1D array=w191, element=w193) -> (index of element=w199:i32)  [unwired: 1 in]
        n117 = case shown="Default" w199 {
          selector: w199 -> [w207 _]
          tunnel: w191 -> [w208 w209]
          tunnel: [w206 w209] -> w196
          frame Default {
            n118 = Delete From Array(array=w208, index=w207) -> (array with subset deleted=w206:string[])  [unwired: 1 in, 1 out]
          }
          frame -1 {
          }
        }
        n119 = Search 1D Array(1D array=w196, element=w190) -> (index of element=w195:i32)  [unwired: 1 in]
        n120 = Max & Min(x=w195, y=0) -> (max(x,y)=w192:i32)  [unwired: 1 out]
        n121 = property on="Frequency" class="LstBox (strict)"("Item Names"=w196, "Value"=w192) -> ()  [unwired: 2 in, 2 out]
      }
      event "Measurement Type": Value Change {
        # "This gets called every time a control changes on the page - keep this in mind"
        # "Hide Tag List?"
        n122 = event-data() -> ()  [unwired: 1 in, 6 out]
        n123 = Unbundle By Name(w211) -> ("Line.Parameters"=w218:T7, "Line.Channel Array"=w213:refnum<class "TBM channel.lvclass">[])
        n124 = Index Array(array=w220, index="Measurement Type") -> (element=w210:T6)
        n125 = case shown="\"Current Input\", \"Current Output\"" w210 {
          selector: w210 -> [_ _ w289 w292 _ _ _]
          tunnel: [w271 w277 w285 w293 w303 w313 w321] -> w217
          tunnel: w218 -> [w270 w276 w283 w291 w302 w312 w320]
          tunnel: [_ TRUE FALSE _ _ _ _] -> w216
          frame "Digital Input", "Digital Output" {
            # "This is currently disabled, because I \ncannot find this property on Create\nChannel, despite it's presence in\nVeristand. I want to keep it here in \nbecause it will be easier to add a new \nproperty later."
            n126 = Bundle By Name(cluster=w270, "Digital Config.Invert Lines?"="Invert Lines?") -> (w271:T7)
            n127 = local write "Tab Control"(T10."Digital" ("Tab Control")) -> ()
            n128 = property on="Invert Lines?" class="Bool (strict)"("Visible"=TRUE) -> ()  [unwired: 2 in, 2 out]
          }
          frame "PWM" {
            n129 = Bundle By Name(cluster=w276, "PWM Config.Idle State"="Idle State") -> (w277:T7)
            n130 = local write "Tab Control"(T1."PWM" ("Tab Control")) -> ()
          }
          frame "Voltage Input", "Voltage Output" {
            n131 = Equal?(x=Measurement_Type."Voltage Input", y=w289) -> (x = y?=w280:bool)
            n132 = Not(x=w280) -> (.not. x?=w281:bool)
            n133 = Bundle By Name(cluster=w283, "Voltage Config.Maximum Value (V)"="Maximum Value (V)", "Voltage Config.Minimum Value (V)"="Minimum Value (V)", "Voltage Config.in terminal configuration (V)"="in terminal configuration (V)", "Voltage Config.out terminal configuration (V)"="out terminal configuration (V)") -> (w285:T7)
            n134 = property on="out terminal configuration (V)" class="Ring (strict)"("Visible"=w281) -> ()  [unwired: 2 in, 2 out]
            n135 = property on="in terminal configuration (V)" class="Ring (strict)"("Visible"=w280) -> ()  [unwired: 2 in, 2 out]
            n136 = local write "Tab Control"(T10."Voltage" ("Tab Control")) -> ()
          }
          frame "Current Input", "Current Output" {
            n137 = Bundle By Name(cluster=w291, "Current Config.Maximum Value (A)"="Maximum Value (A)", "Current Config.Minimum Value (A)"="Minimum Value (A)", "Current Config.shunt resistor location"="shunt resistor location", "Current Config.input terminal configuration (C)"="input terminal configuration (C)", "Current Config.external shunt resistor value"="external shunt resistor value") -> (w293:T7)
            n138 = Equal?(x=Measurement_Type."Current Input", y=w292) -> (x = y?=w300:bool)
            n139 = property on="shunt resistor location" class="Ring (strict)"("Visible"=w300) -> ()  [unwired: 2 in, 2 out]
            n140 = property on="input terminal configuration (C)" class="Ring (strict)"("Visible"=w300) -> ()  [unwired: 2 in, 2 out]
            n141 = property on="external shunt resistor value" class="DigNum (strict)"("Visible"=w300) -> ()  [unwired: 2 in, 2 out]
            n142 = local write "Tab Control"(T10."Current" ("Tab Control")) -> ()
          }
          frame "RTD" {
            n143 = Bundle By Name(cluster=w302, "RTD Config.Maximum Value (°C)"="Maximum Value (°C)", "RTD Config.Minimum Value (°C)"="Minimum Value (°C)", "RTD Config.resistance configuration"="resistance configuration", "RTD Config.r0"="r0", "RTD Config.current excitation value"="current excitation value", "RTD Config.rtd type"="rtd type", "RTD Config.current excitation source"="current excitation source") -> (w303:T7)
            n144 = local write "Tab Control"(T10."RTD" ("Tab Control")) -> ()
          }
          frame "Thermocouple" {
            n145 = Bundle By Name(cluster=w312, "Thermocouple Config.Minimum Value (C)"="Minimum Value (C)", "Thermocouple Config.Maximum Value (C)"="Maximum Value (C)", "Thermocouple Config.thermocouple type"="thermocouple type", "Thermocouple Config.cjc source"="cjc source", "Thermocouple Config.cjc value"="cjc value") -> (w313:T7)
            n146 = local write "Tab Control"(T10."Thermocouple" ("Tab Control")) -> ()
          }
          frame "Strain" {
            n147 = Bundle By Name(cluster=w320, "Strain Config.Maximum Value"="Maximum Value", "Strain Config.Minimum Value"="Minimum Value", "Strain Config.bridge information"="bridge information", "Strain Config.strain gage information"="strain gage information") -> (w321:T7)
            n148 = local write "Tab Control"(T10."Strain" ("Tab Control")) -> ()
          }
        }
        n149 = case shown="\"PWM\"" w210 {
          selector: w210 -> [w232 w252]
          tunnel: [w241 w251] -> w223
          tunnel: w222 -> [w239 w254]
          tunnel: w214 -> [w233 w253]
          tunnel: w211 -> [w230 w248]
          tunnel: w213 -> [w228 w250]
          tunnel: [w226 w249] -> w212
          frame Default {
            n150 = call "Measurement Type to Channel Info.vi"("Measurement Type"=w232) -> ("channel classification"=w234:T11, "Data Type"=w235:T12)  [unwired: 8 in]
            n151 = Index Array(array=w228) -> (element=w227:refnum<class "TBM channel.lvclass">)  [unwired: 1 in]
            n152 = Unbundle By Name(w230) -> ("Maps"=w225:T8[])
            n153 = property class="channel"(reference=w227, error in=w233, "accessors:data type"=w235, "data access:channel classification"=w234) -> (reference out=w224:refnum<class "TBM channel.lvclass">, error out=w242:errorcluster)
            n154 = Index Array(array=w225) -> (element=w231:T8)  [unwired: 1 in]
            n155 = Unbundle By Name(w231) -> ("tag name"=w229:string)
            n156 = call-dynamic "filter tags available for mapping to channel.vi"("channel to map to"=w224, "engine configuration in"=w239) -> ("filtered tags"=w243:refnum<class "tag descriptor.lvclass">[])  [unwired: 8 in, 1 out]
            n157 = for {
              tunnel: w243 -> [w245] mode=indexing
              tunnel: [w244] -> w240 mode=indexing
              n158 = call <vilib>:"read tag name.vi"("system tag in"=w245) -> ("name"=w244:string)  [unwired: 8 in, 2 out]
            }
            n159 = Search 1D Array(1D array=w240, element=w229) -> (index of element=w236:i32)  [unwired: 1 in]
            n160 = Build Array(w224) -> (w226:refnum<class "TBM channel.lvclass">[])
            n161 = Max & Min(x=0 ("f"), y=w236) -> (max(x,y)=w237:i32)  [unwired: 1 out]
            n162 = property on="Tag" class="LstBox (strict)"(error in=w242, "Item Names"=w240, "Val(Sgnl)"=w237) -> (error out=w241:errorcluster)  [unwired: 1 in, 1 out]
          }
          frame "PWM" {
            n163 = Unbundle By Name(w248) -> ("Line.Channel Array"=w247:refnum<class "TBM channel.lvclass">[])
            n164 = Array Size(array=w247) -> (size(s)=w246:i32)
            n165 = case shown="1" w246 {
              tunnel: w254 -> [_ w268]
              tunnel: w253 -> [w255 w267]
              tunnel: w252 -> [_ w266]
              tunnel: w248 -> [_ w265]
              tunnel: [w255 w264] -> w251
              tunnel: w250 -> [w256 w263]
              tunnel: [w256 w262] -> w249
              frame 0, Default {
                # "Only do the initial config if there \nis only 1 channel in the channel array"
              }
              frame 1 {
                n166 = call "generate PWM Tag Lists.vi"("input channel array"=w263, "error in (no error)"=w267, "Mappings in"=w265, "Measurement Type"=w266, "engine configuration in"=w268) -> ("Duty Cycle Index"=w257:i32, "Duty Cycle Array"=w260:string[], "Freq Index"=w258:i32, "Frequency Array"=w261:string[], "output channel array"=w262:refnum<class "TBM channel.lvclass">[])  [unwired: 2 in]
                n167 = property on="Frequency" class="LstBox (strict)"("Item Names"=w261, "Val(Sgnl)"=w258) -> (error out=w259:errorcluster)  [unwired: 2 in, 1 out]
                n168 = property on="Duty Cycle" class="LstBox (strict)"(error in=w259, "Item Names"=w260, "Val(Sgnl)"=w257) -> (error out=w264:errorcluster)  [unwired: 1 in, 1 out]
              }
            }
          }
        }
        n169 = Not(x=w216) -> (.not. x?=w215:bool)
        n170 = Bundle By Name(cluster=w211, "Line.Parameters"=w217, "Line.Channel Array"=w212, "Line.Measurement Type"=w210) -> (w219:T4)
        n171 = property on="Tag" class="LstBox (strict)"("Visible"=w215) -> ()  [unwired: 2 in, 2 out]
      }
    }
    n172 = call "validate line configuration.vi"("Module Config"=w93, "Mappings in"=w102) -> ("valid?"=w99:bool, "errors"=→"errors":string, "Mappings out"=w101:T4)  [unwired: 7 in]
    n173 = Compound Arithmetic op=OR(w105, w100) -> (w104:bool)
    n174 = Select(t=T9."Enabled" ("Disabled"), s=w99, f=T9."Disabled and Grayed Out") -> (s? t:f=w96:T9)
    n175 = property on="ok" class="Bool"("DisabledEnum"=w96) -> ()  [unwired: 2 in, 2 out]
  }
  "success" <- w51
  "Mappings out" <- w45
  n176 = Index Array(array=w8) -> (element #1=w7:refnum<class "TBM channel.lvclass">, element #2=w6:refnum<class "TBM channel.lvclass">)  [unwired: 2 in]
  n177 = call <vilib>:"read tag name.vi"("system tag in"=w7) -> ("name"=w3:string)  [unwired: 8 in, 2 out]
  n178 = call <vilib>:"read tag name.vi"("system tag in"=w6) -> ("name"=w4:string)  [unwired: 8 in, 2 out]
  n179 = Unregister For Events(event registration refnum=w19, error in=w18) -> (error out=w17:errorcluster)
  "error out" <- w17
  n180 = Unbundle By Name(w45) -> ("Line"=w46:T5, "Maps"=w40:T8[])
  n181 = flat-sequence {
    tunnel: w17 -> [_]
    tunnel: w34 -> [w327]
    frame #0 {
      n182 = invoke class="VI" method="FP.Close"(reference=w327) -> ()  [unwired: 2 in, 3 out]
    }
  }
  n183 = Index Array(array=w40) -> (element #1=w39:T8, element #2=w2:T8)  [unwired: 2 in]
  n184 = Unbundle By Name(w39) -> ("tag name"=w38:string)
  n185 = Unbundle By Name(w2) -> ("tag name"=w5:string)
  n186 = Not Equal?(x=w46, y="Line") -> (x != y?=w36:bool)
  n187 = Not Equal?(x=w38, y=w3) -> (x != y?=w37:bool)
  n188 = Not Equal?(x=w5, y=w4) -> (x != y?=w1:bool)
  n189 = Compound Arithmetic op=OR(w36, w37, w1) -> (→"changed":bool)
